vi "Main.vi"(8 "error in (no error)":errorcluster) -> (0 "error out":errorcluster)   [LabVIEW 2017]
uses:
  <vilib>/LVH/i3 JSON/JSON Generation/Create Value Files/Create Value - Object.vi
  <vilib>/LVH/i3 JSON/JSON Generation/Add Object Parameter Files/Add Object Parameter - Numeric.vi
  <vilib>/LVH/i3 JSON/i3-json.lvlib
panel:
  in  "ApiKey":string="1955134594386890752"
  out "OpenTool Json":string
  out "ToolReturn":cluster{"id":string, "result":variant}
  out "Version":cluster{"version":string}
  in  "BaseUrl":string="http://127.0.0.1:8001/opentool"
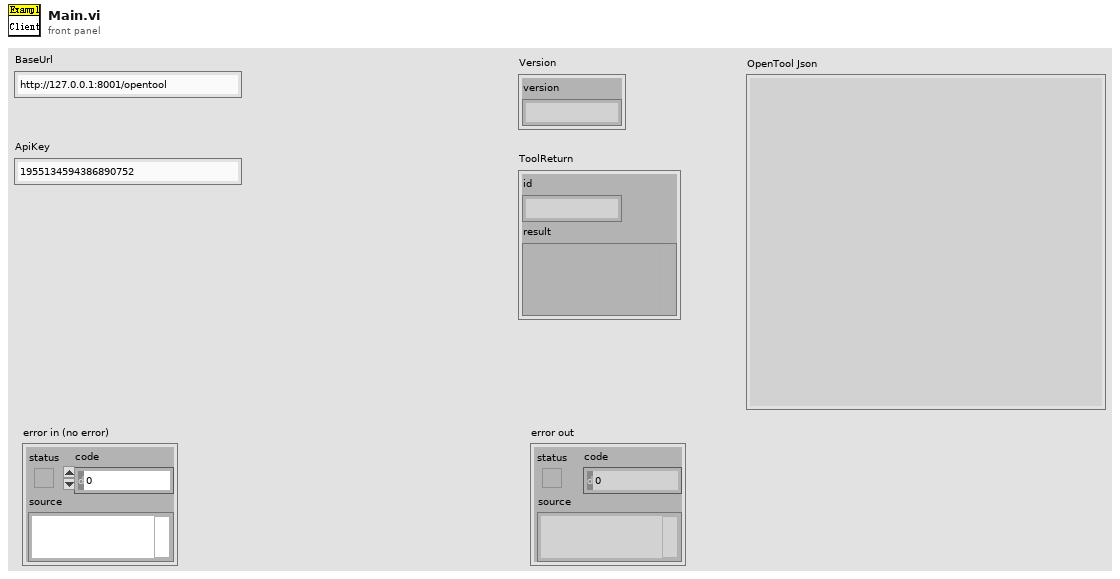
[diagram p1: front panel]
types:
  T1 = cluster{"id":string, "function":string, "arguments":variant}
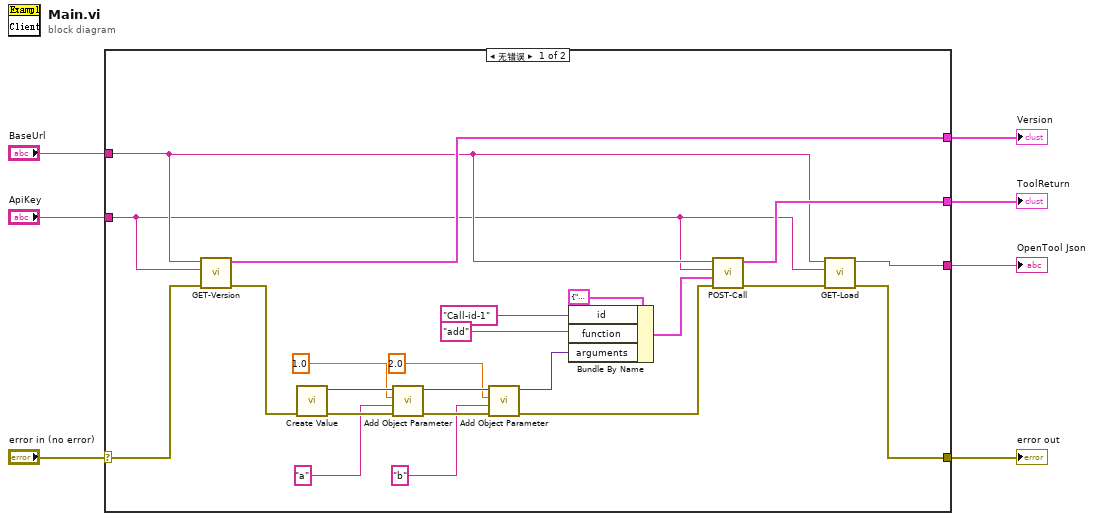
[diagram p0: block diagram]
diagram:
  n1 = case shown="无错误" "error in (no error)" {
    selector: "error in (no error)" -> [w30 w31]
    tunnel: [w28 w31] -> w6
    tunnel: "BaseUrl" -> [w10 _]
    tunnel: [w12 _] -> w4
    tunnel: [w11 _] -> w3
    tunnel: [w8 _] -> w2
    tunnel: "ApiKey" -> [w9 _]
    frame No Error {
      n2 = call "GET-Version.vi"("error in (no error)"=w30, "ApiKey"=w9, "BaseUrl"=w10) -> ("error out"=w14:errorcluster, "Version"=w12:cluster{"version":string})  [unwired: 7 in]
      n3 = call-poly <vilib>:"Create Value.vi"("error in (no error)"=w14) -> ("error out"=w23:errorcluster, "JSON Tree"=w20:variant)  [unwired: 9 in]
      n4 = call-poly <vilib>:"Add Object Parameter.vi"("error in (no error)"=w23, "Name"="a" ("a"), "Numeric"=1.0, "JSON Tree in (JSON Object)"=w20) -> ("error out"=w21:errorcluster, "JSON Tree out (JSON Object)"=w22:variant)  [unwired: 6 in]
      n5 = call-poly <vilib>:"Add Object Parameter.vi"("error in (no error)"=w21, "Name"="b" ("b"), "Numeric"=2.0, "JSON Tree in (JSON Object)"=w22) -> ("error out"=w13:errorcluster, "JSON Tree out (JSON Object)"=w15:variant)  [unwired: 6 in]
      n6 = Bundle By Name(cluster=T1 {"id"="", "function"="", "arguments"=variant} ("FunctionCall"), "id"="Call-id-1", "function"="add", "arguments"=w15) -> (w26:T1)
      n7 = call "POST-Call.vi"("error in (no error)"=w13, "FunctionCall"=w26, "ApiKey"=w9, "BaseUrl"=w10) -> ("error out"=w29:errorcluster, "ToolReturn"=w11:cluster{"id":string, "result":variant})  [unwired: 6 in]
      n8 = call "GET-Load.vi"("error in (no error)"=w29, "ApiKey"=w9, "BaseUrl"=w10) -> ("error out"=w28:errorcluster, "OpenTool Json"=w8:string)  [unwired: 7 in]
    }
    frame Error {
    }
  }
  "error out" <- w6
  "Version" <- w4
  "ToolReturn" <- w3
  "OpenTool Json" <- w2
